vi "CloseHandle Wrapper Template.vi"(0 "hObject":u64, 11 "error in":errorcluster) -> (4 "return value":i32, 15 "error out":errorcluster)   [LabVIEW 2020]
doc: "Closes a kernel object handle (here, one kernel32 OpenProcess.vi returned) through kernel32.dll CloseHandle (stdcall, called in any thread). return value is the Win32 BOOL: non-zero on success. When error in carries an error the DLL is not called. Generated by scripts\\Build Win32 Wrappers.vi - do not edit by hand, rebuild it."
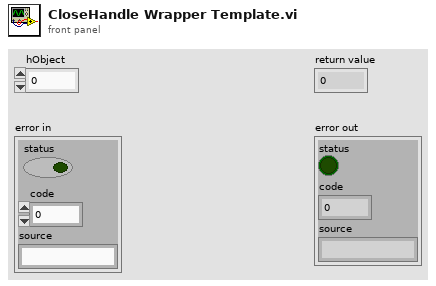
[diagram p1: front panel]
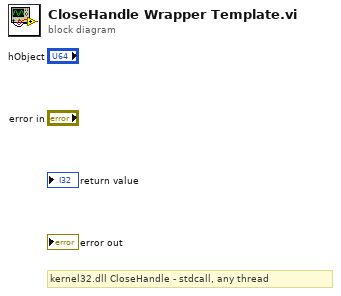
[diagram p0: block diagram]
diagram:
  # "kernel32.dll CloseHandle - stdcall, any thread"
